vi "导出扫描测试数据.vi"(6 "导出数据选择":enum8{"False", "True", "Mixed"}(c332), 11 "数据":T1[](array[typedef])) -> (2 "突变电压":dbl[][](array[numeric]), 3 "扫描数据":dbl[][](array[numeric]))   [LabVIEW 2020]
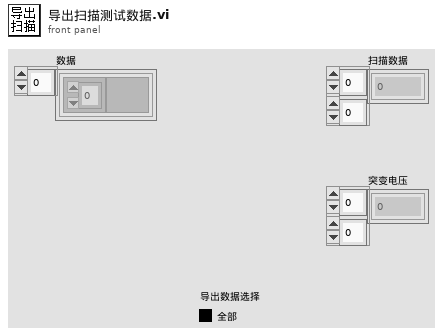
[diagram p1: front panel]
types:
  T1 = typedef "数据显示.xctl/波形数据定义.ctl" = cluster{"波形":dbl[][], "属性":variant}
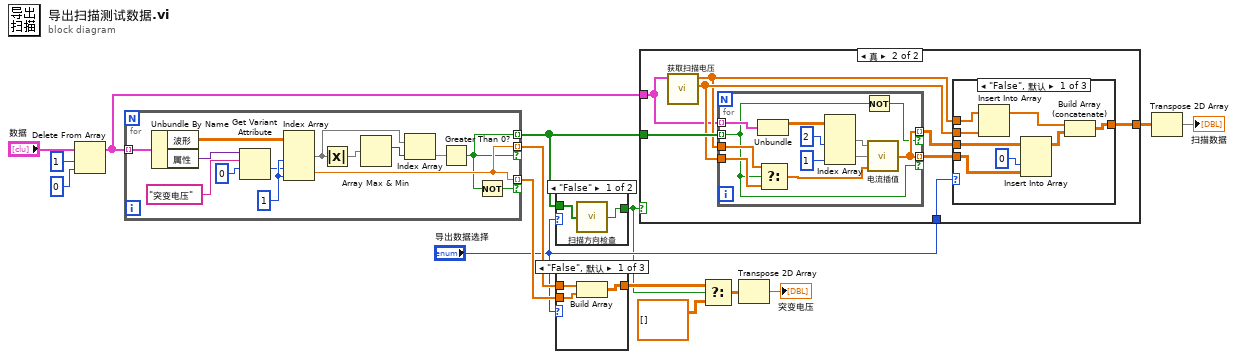
[diagram p0: block diagram]
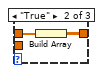
[diagram p2: hidden frame]
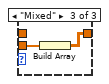
[diagram p3: hidden frame]
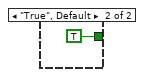
[diagram p4: hidden frame]
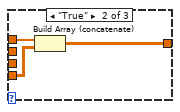
[diagram p6: hidden frame]
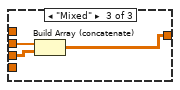
[diagram p7: hidden frame]
diagram:
  n1 = Delete From Array(array="数据", length=1 ("长度"), index=0 ("索引")) -> (array with subset deleted=w6:T1[])  [unwired: 1 out]
  n2 = for {
    tunnel: w6 -> [w29] mode=indexing
    tunnel: [w21] -> w13 mode=indexing if=w20
    tunnel: [w20] -> w15 mode=indexing
    tunnel: [w21] -> w12 mode=indexing if=w16
    w24 = 1 ("禁用的索引 (列)")
    n3 = Unbundle By Name(w29) -> ("波形"=w25:dbl[][], "属性"=w28:variant)
    n4 = Get Variant Attribute(Variant=w28, name="突变电压" ("名称"), default value (empty Variant)=0 ("突变电压")) -> (value=w23:i32)  [unwired: 1 in, 3 out]
    n5 = Index Array(array=w25, index (col) #1=w24, index (row) #2=w23, index (col) #2=w24) -> (element #1=w18:dbl[], element #2=w21:dbl)  [unwired: 1 in]
    n6 = Absolute Value(x=w18) -> (abs(x)=w19:dbl[])
    n7 = Array Max & Min(array=w19) -> (max index (indices)=w17:i32)  [unwired: 3 out]
    n8 = Index Array(array=w18, index=w17) -> (element=w22:dbl)
    n9 = Greater Than 0?(x=w22) -> (x > 0?=w20:bool)
    n10 = Not(x=w20) -> (.not. x?=w16:bool)
  }
  n11 = case shown="\"False\"" "导出数据选择" {
    tunnel: w15 -> [w31 _]
    tunnel: [w30 TRUE ("检查通过？")] -> w4
    frame "False" {
      n12 = call "扫描方向检查.vi"("扫描方向"=w31) -> ("检查通过？"=w30:bool)
    }
    frame "True", Default {
    }
  }
  n13 = case shown="\"False\", 默认" "导出数据选择" {
    tunnel: w13 -> [w35 w37 _]
    tunnel: w12 -> [w34 _ w38]
    tunnel: [w33 w36 w39] -> w11
    frame "False", Default {
      n14 = Build Array(w35, w34) -> (w33:dbl[][])
    }
    frame "True" {
      n15 = Build Array(w37) -> (w36:dbl[][])
    }
    frame "Mixed" {
      n16 = Build Array(w38) -> (w39:dbl[][])
    }
  }
  n17 = case shown="真" w4 {
    tunnel: w15 -> [_ w47]
    tunnel: [_ w46] -> w14
    tunnel: "导出数据选择" -> [_ w45]
    tunnel: w6 -> [_ w40]
    frame False {
    }
    frame True {
      n18 = call "获取扫描电压.vi"("数据"=w40) -> ("负"=w42:dbl[], "正"=w41:dbl[])  [unwired: 9 in]
      n19 = for {
        tunnel: w40 -> [w73] mode=indexing
        tunnel: w47 -> [w65] mode=indexing
        tunnel: w41 -> [w68]
        tunnel: w42 -> [w67]
        tunnel: [w66] -> w44 mode=indexing if=w65
        tunnel: [w66] -> w43 mode=indexing if=w64
        n20 = Unbundle(w73) -> ("波形"=w72:dbl[][])  [unwired: 1 out]
        n21 = Select(t=w68, s=w65, f=w67) -> (s? t:f=w69:dbl[])
        n22 = Index Array(array=w72, index (col) #1=2 ("索引 (行)"), index (col) #2=1 ("索引 (行)")) -> (element #1=w71:dbl[], element #2=w70:dbl[])  [unwired: 2 in]
        n23 = Not(x=w65) -> (.not. x?=w64:bool)
        n24 = call "电流插值.vi"("电压"=w69, "原始电压"=w70, "原始电流"=w71) -> ("插值后电流"=w66:dbl[])
      }
      n25 = case shown="\"False\", 默认" w45 {
        tunnel: w41 -> [w55 w58 _]
        tunnel: w42 -> [w54 _ w60]
        tunnel: w44 -> [w53 w56 _]
        tunnel: w43 -> [w51 _ w59]
        tunnel: [w48 w57 w61] -> w46
        frame "False", Default {
          n26 = Insert Into Array(array=w55, new element=w54) -> (w50:dbl[])  [unwired: 1 in]
          n27 = Insert Into Array(array=w51, index (col)=0 ("索引 (列)"), new element=w53) -> (w49:dbl[][])  [unwired: 1 in]
          n28 = Build Array (concatenate)(w50, w49) -> (w48:dbl[][])
        }
        frame "True" {
          n29 = Build Array (concatenate)(w58, w56) -> (w57:dbl[][])
        }
        frame "Mixed" {
          n30 = Build Array (concatenate)(w60, w59) -> (w61:dbl[][])
        }
      }
    }
  }
  n31 = Select(t=w11, s=w4, f=dbl[][] []) -> (s? t:f=w5:dbl[][])
  n32 = Transpose 2D Array(2D array=w5) -> (transposed array=→"突变电压":dbl[][])
  n33 = Transpose 2D Array(2D array=w14) -> (transposed array=→"扫描数据":dbl[][])
